vi "Test TDMS Read Speed.vi"(8 "error in (no error)":errorcluster, 11 "Path":path) -> (0 "error out":errorcluster, 2 "time (ms/file)":u32, 3 "dup Folder Path":path)   [LabVIEW 2019]
uses:
  LV-Data/LV-Data.lvclass
panel:
  in  "stop":bool
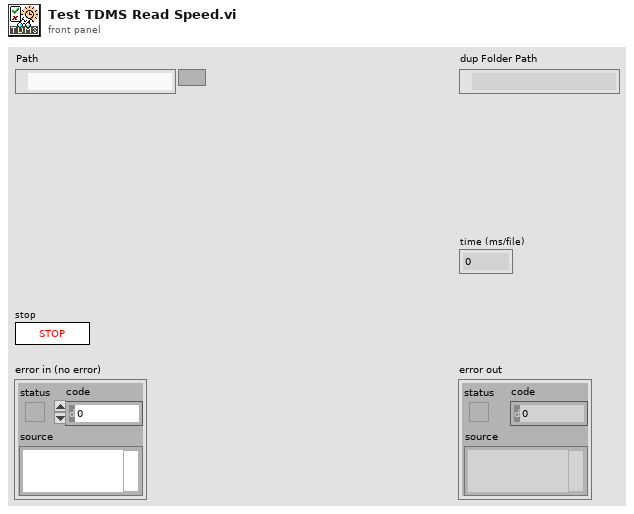
[diagram p1: front panel]
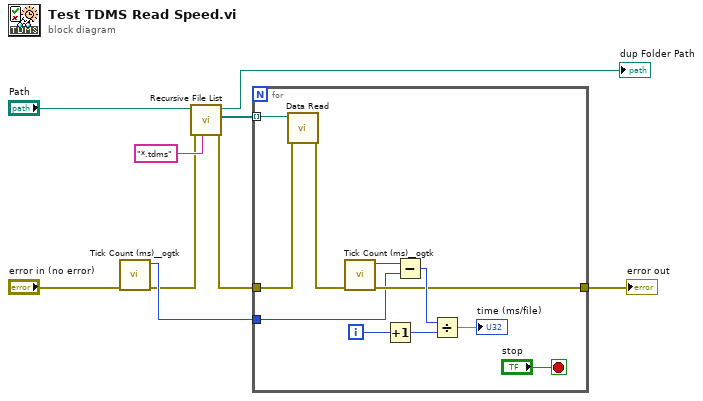
[diagram p0: block diagram]
diagram:
  n1 = call <userlib>:"Tick Count (ms)__ogtk.vi"("error in (no error)"="error in (no error)") -> ("error out"=w3:errorcluster, "millisecond timer value"=w5:u32)  [unwired: 9 in]
  n2 = call <vilib>:"Recursive File List.vi"("pattern"="*.tdms", "error in (no error)"=w3, "Folder Path"="Path") -> ("error out"=w2:errorcluster, "All Files in Dir"=w6:path[], "dup Folder Path"=→"dup Folder Path":path)  [unwired: 4 in, 2 out]
  n3 = for {
    tunnel: w6 -> [w12] mode=indexing
    tunnel: w2 -> [w11]
    tunnel: [w14] -> w4
    tunnel: w5 -> [w13]
    i -> [w19]
    stop <- "stop" stop-if-true
    n4 = call "Data Read.vi"("error in (no error)"=w11, "path"=w12) -> ("error out"=w10:errorcluster)  [unwired: 6 in, 3 out]
    n5 = call <userlib>:"Tick Count (ms)__ogtk.vi"("error in (no error)"=w10) -> ("error out"=w14:errorcluster, "millisecond timer value"=w15:u32)  [unwired: 9 in]
    n6 = Increment(x=w19) -> (x+1=w18:i32)
    n7 = Subtract(x=w15, y=w13) -> (x-y=w20:u32)
    n8 = Divide(x=w20, y=w18) -> (x/y=→"time (ms/file)":dbl)
  }
  "error out" <- w4
